vi "Close.vi"(8 "error in (no error)":errorcluster, 11 "channel in":refnum<class "CANsub_DirectChannel.lvclass">) -> (0 "error out":errorcluster, 3 "channel out":refnum<class "CANsub_DirectChannel.lvclass">)   [LabVIEW 2021, in "CANsub_API.lvlib" / "CANsub_DirectChannel.lvclass"]
doc: "Direct: if the channel is Open or Lost, closes it with C7 (WebSocket close, DELETE /ws fallback); state = Closed. Runs also with an error in; the original error comes first. Setup/teardown only: do not call in a periodic loop (allocates, may block)."
uses:
  CANsub_DirectChannel.lvclass
  CANsub_DirectChannel.lvclass/CANsub_DirectChannel.ctl
  common/CANsub_Common.lvlib
  Typedefs/CANsub_State.ctl
  CANsub_API.lvlib
  <vilib>/httpClient/ClientHandle.ctl
  <vilib>/httpClient/LabVIEWHTTPClient.lvlib
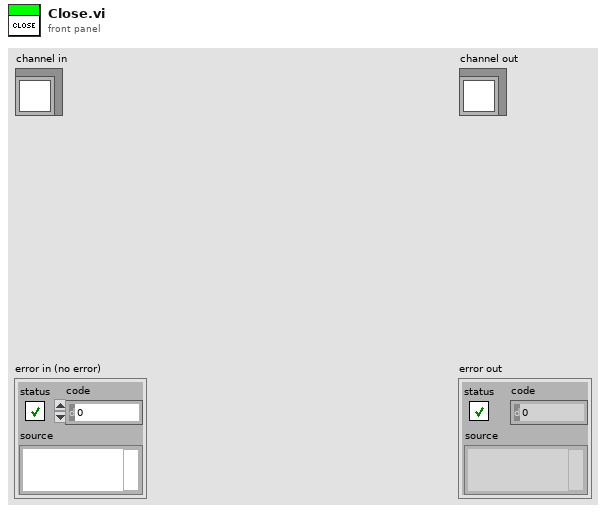
[diagram p1: front panel]
types:
  T1 = typedef "CANsub_API.lvlib/CANsub_State.ctl" = enum16{"Closed", "Open", "Lost"}
  T2 = typedef "LabVIEWHTTPClient.lvlib/ClientHandle.ctl" = refnum<k1>
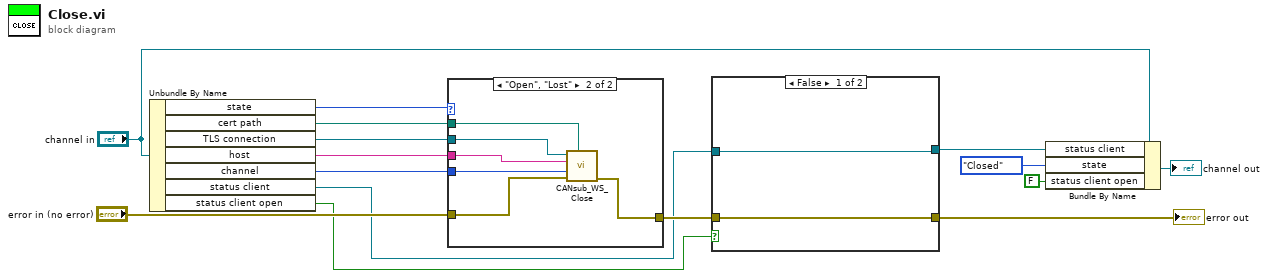
[diagram p0: block diagram]
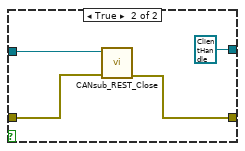
[diagram p2: hidden frame]
diagram:
  n1 = Unbundle By Name("channel in") -> ("state"=w15:T1, "cert path"=w13:path, "TLS connection"=w12:refnum<k5>, "host"=w11:string, "channel"=w10:u8, "status client"=w3:T2, "status client open"=w6:bool)
  n2 = case shown="\"Open\", \"Lost\"" w15 {
    tunnel: "error in (no error)" -> [w16 w22]
    tunnel: w13 -> [_ w21]
    tunnel: w12 -> [_ w20]
    tunnel: w11 -> [_ w19]
    tunnel: w10 -> [_ w18]
    tunnel: [w16 w17] -> w5
    frame "Closed", Default {
    }
    frame "Open", "Lost" {
      n3 = call "CANsub_WS_Close.vi"("cert path"=w21, "error in (no error)"=w22, "channel"=w18, "host"=w19, "TLS Connection"=w20) -> ("error out"=w17:errorcluster)  [unwired: 5 in, 1 out]
    }
  }
  n4 = case shown="False" w6 {
    tunnel: w5 -> [w24 w28]
    tunnel: [w24 w27] -> w4
    tunnel: w3 -> [w23 w26]
    tunnel: [w23 T2 refnum ("status client")] -> w1
    frame False {
    }
    frame True {
      n5 = call "CANsub_REST_Close.vi"("error in (no error)"=w28, "client handle"=w26) -> ("error out"=w27:errorcluster)  [unwired: 9 in]
    }
  }
  "error out" <- w4
  n6 = Bundle By Name(cluster="channel in", "status client"=w1, "state"=CANsub_State."Closed" ("status.state"), "status client open"=FALSE) -> (→"channel out":refnum<class "CANsub_DirectChannel.lvclass">)
